vi "MemoryMapMain.vi"(8 "error in (no error)":errorcluster, 11 "MemoryMap in":refnum<class "MemoryMap.lvclass">) -> (3 "MemoryMap out":refnum<class "MemoryMap.lvclass">)   [LabVIEW 2020, in "Sgraph_lib_V1.lvlib" / "MemoryMap.lvclass"]
uses:
  MemoryMap.lvclass
  Gserver/controls/Typedef_Gviewer-Query.ctl
  Gserver/controls/Typedef_QueryType.ctl
  Common/controls/MeMapInfo.ctl
  Common/controls/MMap_element.ctl
  Builds/Sgraph_lib_V1.lvlib
  Gserver/Gserver.lvclass
panel:
  in  "Layer":i32 min=0 max=6
  out "Graph 3":cluster{"Array":dbl[]}[](graph)
  out "Graph 2":cluster{"Array":dbl[]}[](graph)
  out "Graph 1":cluster{"Array":dbl[]}[](graph)
  out "37x37":picture
  in  "Gserver-Queue":refnum<queue>
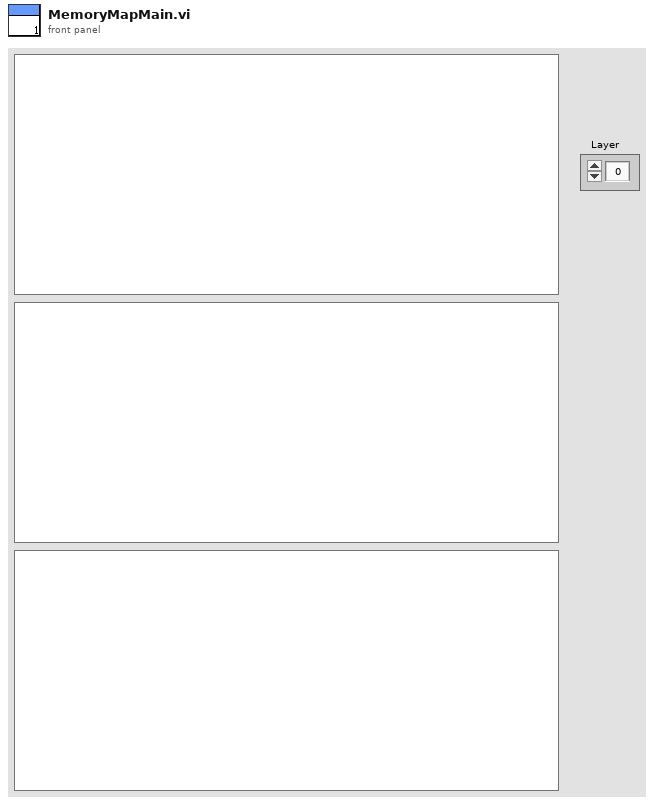
[diagram p1: front panel]
types:
  T1 = typedef "Sgraph_lib_V1.lvlib/MeMapInfo.ctl" = cluster{"MemLayer":T2[]}
  T2 = typedef "Sgraph_lib_V1.lvlib/MMap_element.ctl" = cluster{"Name":string, "Length":i32, "Pointer":i32, "Tbegin":dbl, "Tend":dbl, "Tmin":dbl, "Tmax":dbl, "Tpnt-1":dbl, "Tpnt":dbl, "Tpnt+1":dbl, "Array":dbl[]}
  T3 = typedef "LVBoundsTypeDef.ctl" = cluster{"Width":u32, "Height":u32}
  T4 = typedef "Sgraph_lib_V1.lvlib/Gserver.lvclass/Typedef_QueryType.ctl" = enum16{"Subscribe", "DataRequest", "RequestAllTags", "RequestIniPath", "FAMMstarted", "SetClientOptions", "GviewerUpdate", "OpenNewGraph", "CloseClient", "CloseAllClients", "Close Gserver", "OpenMemoryMap", "MeMapDataRequest", "MeMapDataResponse"}
  T5 = typedef "Sgraph_lib_V1.lvlib/Gserver.lvclass/Typedef_Gviewer-Query.ctl" = cluster{"Query_type":T4, "data":variant, "Source":string, "Time Stamp":timestamp}
  T6 = cluster{"horizontal":enum16{"left", "center", "right"}, "vertical":enum16{"top", "center", "bottom"}}
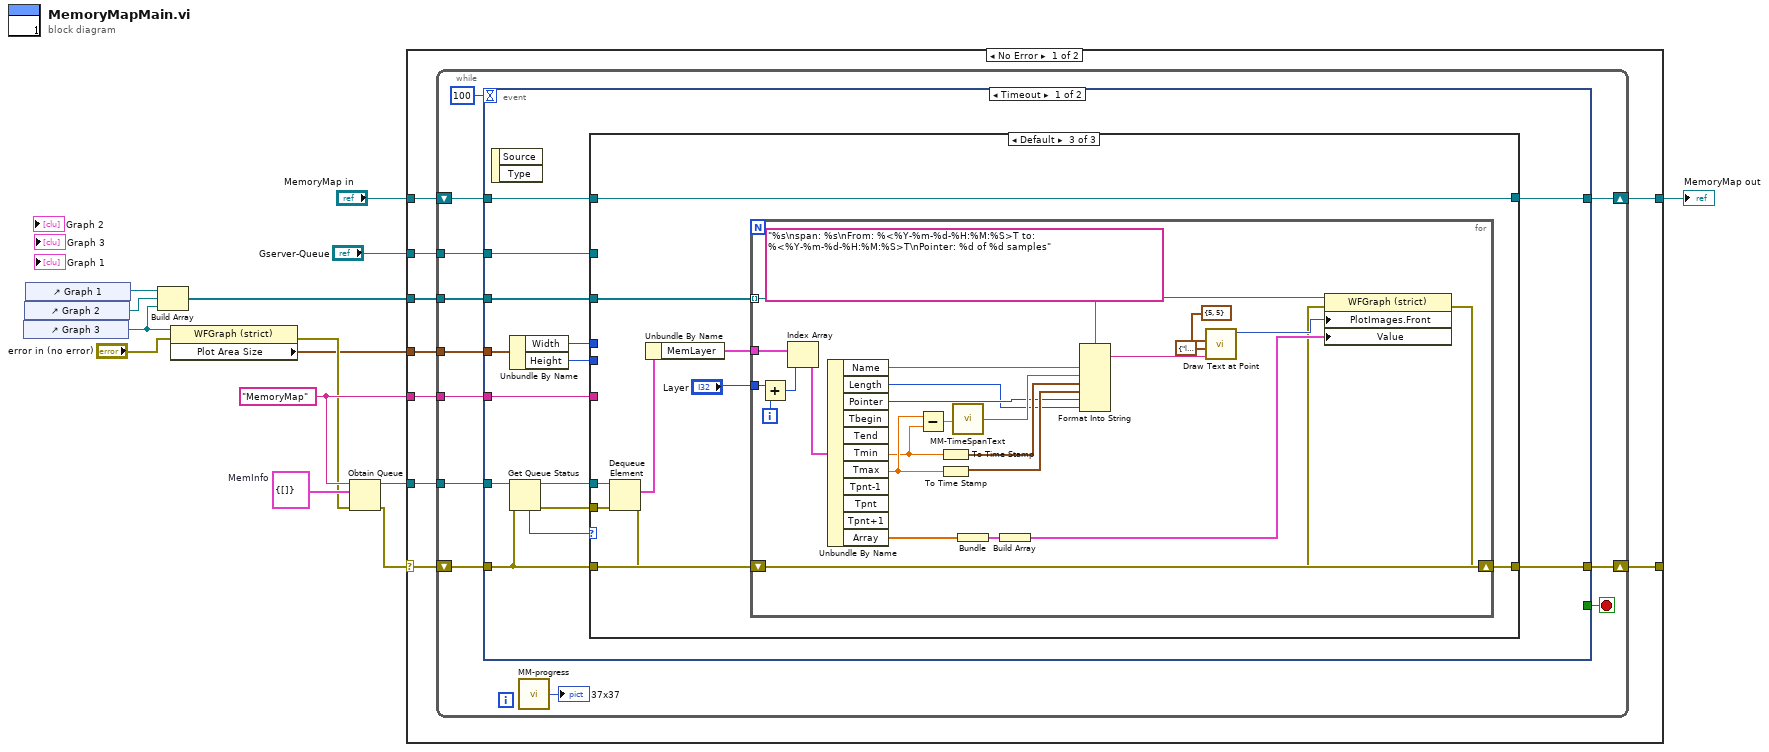
[diagram p0: block diagram]
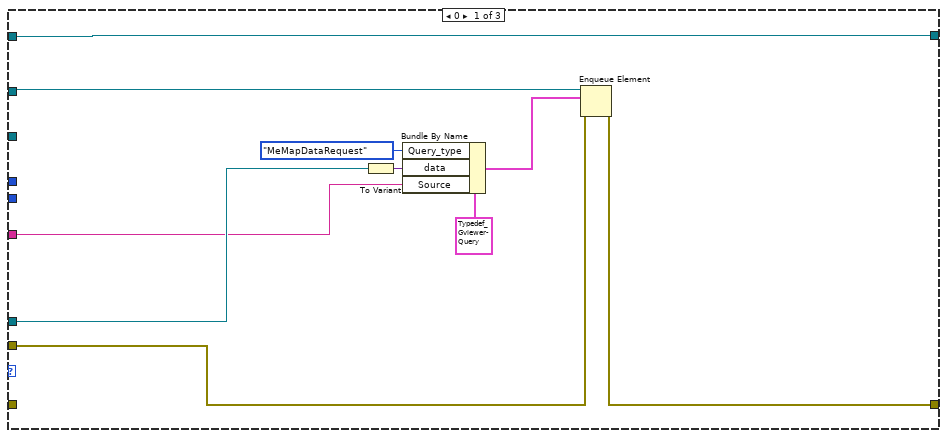
[diagram p2: hidden frame]
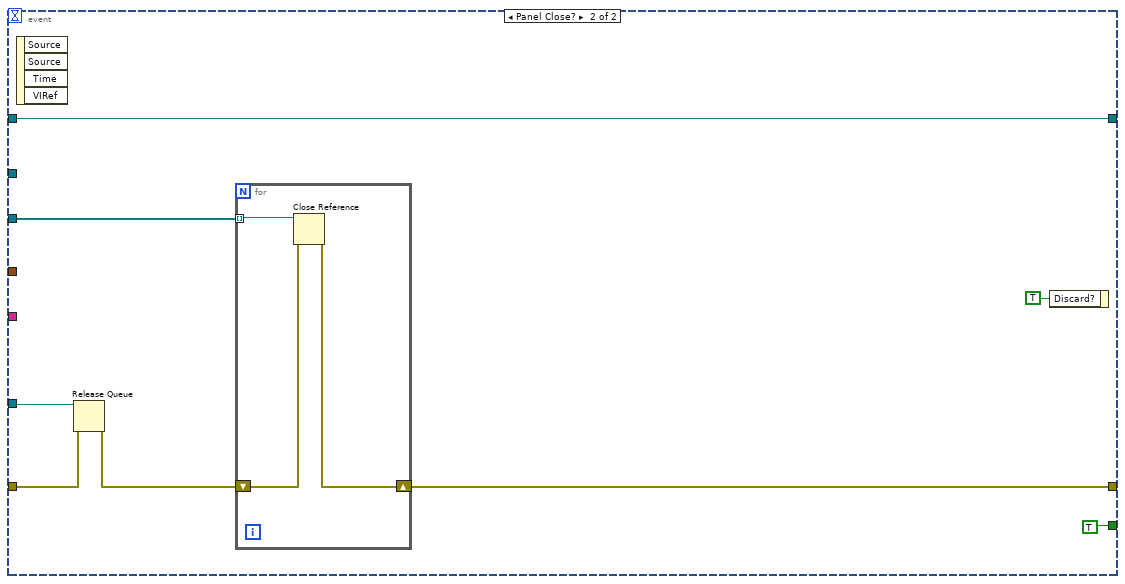
[diagram p4: hidden frame]
diagram:
  w8 = "MemoryMap" ("name (unnamed)")
  w11 = T1 {"MemLayer"=[]}  # MemInfo
  n1 = control-ref of="Graph 3"() -> (w4:refnum<vi>)
  n2 = control-ref of="Graph 2"() -> (w5:refnum<vi>)
  n3 = control-ref of="Graph 1"() -> (w6:refnum<vi>)
  n4 = Build Array(w6, w5, w4) -> (w7:refnum<vi>[])
  n5 = property class="WFGraph (strict)"(reference=w4, error in="error in (no error)") -> (error out=w2:errorcluster, "Plot Area Size"=w1:T3)  [unwired: 1 out]
  n6 = Obtain Queue(name (unnamed)=w8, element data type=w11, error in (no error)=w2) -> (queue out=w9:refnum<queue>, error out=w10:errorcluster)  [unwired: 2 in, 1 out]
  n7 = case shown="No Error" w10 {
    selector: w10 -> [w21 w106]
    tunnel: [w21 w106] -> _
    tunnel: [w20 w105] -> w13
    tunnel: "MemoryMap in" -> [w20 w105]
    tunnel: "Gserver-Queue" -> [w19 _]
    tunnel: w9 -> [w18 _]
    tunnel: w8 -> [w17 _]
    tunnel: w7 -> [w16 _]
    tunnel: w1 -> [w15 _]
    frame No Error {
      n8 = while {
        shift-right: [w30] -> _
        shift-left: w20 -> [w32]
        shift-right: [w29] -> _
        shift-left: w21 -> [w31]
        tunnel: w19 -> [w28]
        tunnel: w18 -> [w27]
        tunnel: w17 -> [w26]
        tunnel: w16 -> [w25]
        tunnel: w15 -> [w22]
        stop <- w23 stop-if-true
        n9 = event shown="[0] Timeout" {
          selector: _ -> [_ _]
          dyn-events: _ -> [_ _]
          timeout: 100 -> [_ _]
          tunnel: w32 -> [w47 w99]
          tunnel: w31 -> [w34 w97]
          tunnel: [w46 w99] -> w30
          tunnel: [w45 w95] -> w29
          tunnel: w28 -> [w36 _]
          tunnel: w27 -> [w44 w98]
          tunnel: w26 -> [w35 _]
          tunnel: w25 -> [w43 w94]
          tunnel: [_ TRUE] -> w23
          tunnel: w22 -> [w39 _]
          event Timeout {
            n10 = event-data() -> ()  [unwired: 1 in, 2 out]
            n11 = Unbundle By Name(w39) -> ("Width"=w38:u32, "Height"=w37:u32)
            n12 = Get Queue Status(queue=w44, error in (no error)=w34) -> (queue out=w40:refnum<queue>, error out=w41:errorcluster, # elements in queue=w42:i32)  [unwired: 1 in, 5 out]
            n13 = case shown="Default" w42 {
              tunnel: w47 -> [w57 w58 w68]
              tunnel: [w57 w58 w68] -> w46
              tunnel: w41 -> [w48 _ w66]
              tunnel: [w49 w59 w61] -> w45
              tunnel: w40 -> [w53 _ w67]
              tunnel: w43 -> [_ _ w63]
              tunnel: w38 -> [_ _ _]
              tunnel: w37 -> [_ _ _]
              tunnel: w36 -> [w56 _ _]
              tunnel: w35 -> [w51 _ _]
              tunnel: w34 -> [_ w59 _]
              frame 0 {
                n14 = To Variant(anything=w53) -> (Variant=w52:variant)
                n15 = Bundle By Name(cluster=T5 {"Query_type"=enum."MeMapDataRequest", "data"=variant, "Source"="", "Time Stamp"=timestamp(0 s since 1904-01-01)} ("element"), "Query_type"=Typedef_QueryType."MeMapDataRequest", "data"=w52, "Source"=w51) -> (w50:T5)
                n16 = Enqueue Element(queue=w56, element=w50, error in (no error)=w48) -> (error out=w49:errorcluster)  [unwired: 1 in, 2 out]
              }
              frame -1 {
              }
              frame Default {
                n17 = Dequeue Element(queue=w67, error in (no error)=w66) -> (element=w65:T1, error out=w62:errorcluster)  [unwired: 1 in, 2 out]
                n18 = Unbundle By Name(w65) -> ("MemLayer"=w64:T2[])
                n19 = for {
                  tunnel: w64 -> [w84]
                  tunnel: w63 -> [w85] mode=indexing
                  shift-right: [w86] -> w61
                  shift-left: w62 -> [w87]
                  tunnel: "Layer" -> [w73]
                  i -> [w72]
                  n20 = Add(x=w73, y=w72) -> (x+y=w71:i32)
                  n21 = Index Array(array=w84, index=w71) -> (element=w83:T2)
                  n22 = Unbundle By Name(w83) -> ("Name"=w82:string, "Length"=w69:i32, "Pointer"=w70:i32, "Tmin"=w74:dbl, "Tmax"=w79:dbl, "Array"=w93:dbl[])  [unwired: 5 out]
                  n23 = Subtract(x=w79, y=w74) -> (x-y=w78:dbl)
                  n24 = To Time Stamp(1:w74) -> (0:w76:timestamp)
                  n25 = To Time Stamp(1:w79) -> (0:w75:timestamp)
                  n26 = call "MM-TimeSpanText.vi"("Timespan"=w78) -> ("TimeSpanText"=w77:string)  [unwired: 4 in]
                  n27 = Bundle("Array"=w93) -> (w89:cluster{"Array":dbl[]})  [unwired: 1 in]
                  n28 = Build Array(w89) -> (w88:cluster{"Array":dbl[]}[])
                  n29 = Format Into String(format string="%s\nspan: %s\nFrom: %<%Y-%m-%d-%H:%M:%S>T to: %<%Y-%m-%d-%H:%M:%S>T\nPointer: %d of %d samples", w82, w77, w76, w75, w70, w69) -> (resulting string=w81:string)  [unwired: 2 in, 1 out]
                  n30 = call <vilib>:"Draw Text at Point.vi"("text"=w81, "alignment(left, top)"=T6 {"horizontal"=enum."left", "vertical"=enum."top"}, "origin"=cluster{"x":i16, "y":i16} {"x"=5, "y"=5}) -> ("new picture"=w90:picture)  [unwired: 7 in, 1 out]
                  n31 = property class="WFGraph (strict)"(reference=w85, error in=w87, "PlotImages.Front"=w90, "Value"=w88) -> (error out=w86:errorcluster)  [unwired: 1 out]
                }
              }
            }
          }
          event Panel Close? {
            n32 = event-data() -> ()  [unwired: 1 in, 4 out]
            n33 = Release Queue(queue=w98, error in (no error)=w97) -> (error out=w96:errorcluster)  [unwired: 1 in, 2 out]
            n34 = for {
              shift-right: [w102] -> w95
              shift-left: w96 -> [w103]
              tunnel: w94 -> [w104] mode=indexing
              n35 = Close Reference(reference=w104, error in (no error)=w103) -> (error out=w102:errorcluster)
            }
            n36 = event-data("Discard?"=TRUE) -> ()  [unwired: 1 in, 1 out]
          }
        }
        n37 = call "MM-progress.vi"() -> ("37x37"=→"37x37":picture)  [unwired: 7 in]
      }
    }
    frame Error {
    }
  }
  "MemoryMap out" <- w13
